vi "TCP Server Search Connections for Connection.vi"(3 "Connections":T1[](array[typedef]), 4 "dup connection IDs (for quick search)":refnum<k5>[](array[refnum]), 5 "connection ID":refnum<k5>) -> (0 "index":i32, 1 "Found?":bool, 2 "Connection Info":T1)   [LabVIEW 2020, in "JKI TCP Server.lvclass"]
uses:
  JKI TCP Server.lvclass
  _Data Structures/TCP Server Connection Info Cluster.ctl
panel:
  # "Copyright © 2004-2008 JKI. All rights reserved.\n\nAuthor: Jim Kring [jim.kring@jameskring.com]\n\nThis library is provided \"AS IS\" ,WITHOUT WARRANTIES OR \nCONDITIONS OF ANY KIND, either express or implied.\n\nJames Kring, Inc. -- http://www.jameskring.com"
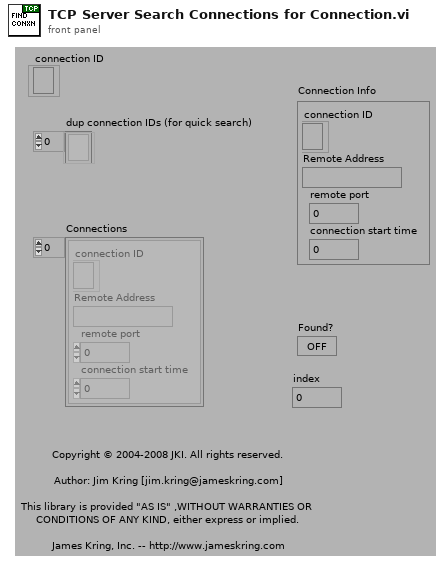
[diagram p1: front panel]
types:
  T1 = typedef "JKI TCP Server.lvclass/TCP Server Connection Info Cluster.ctl" = cluster{"connection ID":refnum<k5>, "Remote Address":string, "remote port":u16, "connection start time":u32}
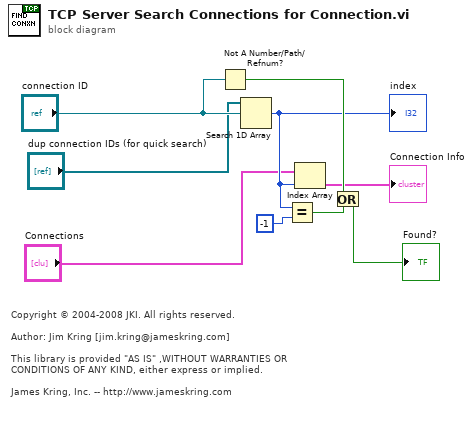
[diagram p0: block diagram]
diagram:
  # "Copyright © 2004-2008 JKI. All rights reserved.\n\nAuthor: Jim Kring [jim.kring@jameskring.com]\n\nThis library is provided \"AS IS\" ,WITHOUT WARRANTIES OR \nCONDITIONS OF ANY KIND, either express or implied.\n\nJames Kring, Inc. -- http://www.jameskring.com"
  n1 = Not A Number/Path/Refnum?(number/path/refnum="connection ID") -> (NaN/Path/Refnum?=w8:bool)
  n2 = Search 1D Array(1D array="dup connection IDs (for quick search)", element="connection ID") -> (index of element=w3:i32)  [unwired: 1 in]
  "index" <- w3
  n3 = Equal?(x=w3, y=-1) -> (x = y?=w6:bool)
  n4 = Index Array(array="Connections", index=w3) -> (element=→"Connection Info":T1)
  n5 = Or(x=w8, y=w6) -> (x .or. y?=→"Found?":bool)
